vi "Is Object Selected.vi"(9 "error in (no error)":errorcluster, 10 "GObject Reference":refnum<vi>) -> (1 "error out":errorcluster, 2 "Selected":bool)   [LabVIEW 2012, in "Scripting Tools.lvlib"]
doc: "Is the <b>GObject Reference</b> selected in the editor or not ?"
uses:
  Scripting Tools.lvlib
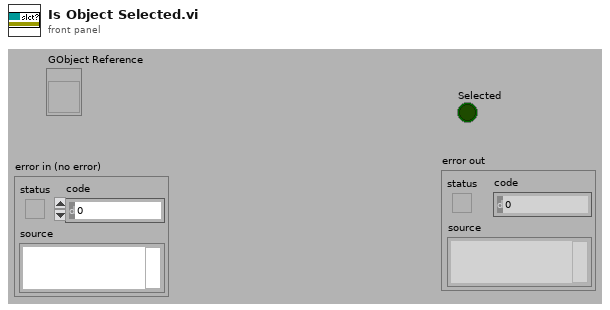
[diagram p1: front panel]
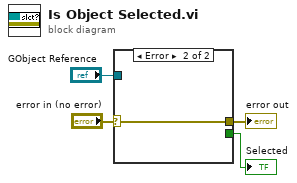
[diagram p0: block diagram]
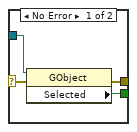
[diagram p2: hidden frame]
diagram:
  n1 = case shown="Error" "error in (no error)" {
    selector: "error in (no error)" -> [w8 w9]
    tunnel: [w7 w9] -> w3
    tunnel: "GObject Reference" -> [w6 _]
    tunnel: [w5 _] -> w1
    frame No Error {
      n2 = property class="GObject"(reference=w6, error in=w8) -> (error out=w7:errorcluster, "Selected"=w5:bool)  [unwired: 1 out]
    }
    frame Error {
    }
  }
  "error out" <- w3
  "Selected" <- w1
